vi "kernel32 CloseHandle.vi"(0 "hObject":u64, 11 "error in":errorcluster) -> (4 "return value":i32, 15 "error out":errorcluster)   [LabVIEW 2020, in "RemoteVI.lvlib"]
doc: "Closes a kernel object handle (here, one kernel32 OpenProcess.vi returned) through kernel32.dll CloseHandle (stdcall, called in any thread). return value is the Win32 BOOL: non-zero on success. When error in carries an error the DLL is not called. Generated by scripts\\Build Win32 Wrappers.vi - do not edit by hand, rebuild it."
uses:
  RemoteVI.lvlib
  kernel32.dll
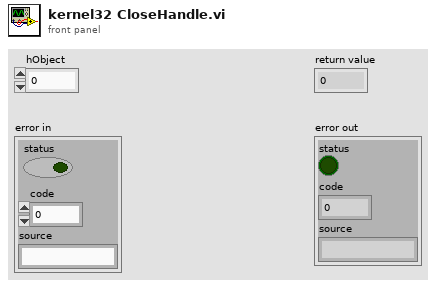
[diagram p1: front panel]
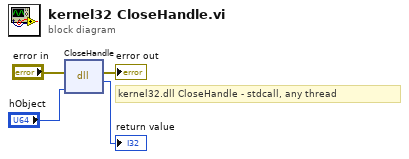
[diagram p0: block diagram]
diagram:
  # "kernel32.dll CloseHandle - stdcall, any thread"
  n1 = dll-call lib="kernel32.dll" fn="CloseHandle"(error in="error in", "hObject"="hObject") -> (error out=→"error out":errorcluster, →"return value":i32)  [unwired: 3 in, 1 out]
